vi "set OBW - Sweep Time.vi"(8 "error in (no error)":errorcluster, 9 "Auto?":bool, 10 "Sweep Time (s)":dbl format="%#_6p", 11 "Keysight 9020A in":refnum<class "Keysight 9020A.lvclass">) -> (0 "error out":errorcluster, 3 "Keysight 9020A out":refnum<class "Keysight 9020A.lvclass">)   [LabVIEW 2023, in "Spectrum Analyzer.lvlib" / "Keysight 9020A.lvclass"]
uses:
  Keysight 9020A.lvclass
  Keysight 9020A.lvclass/Keysight 9020A.ctl
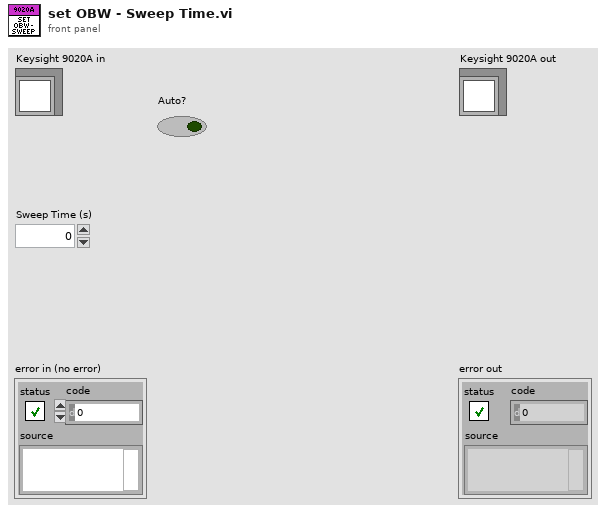
[diagram p1: front panel]
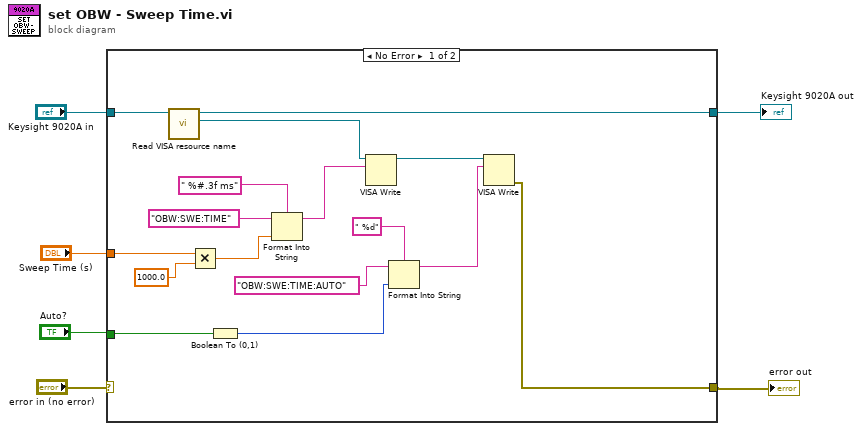
[diagram p0: block diagram]
diagram:
  n1 = case shown="No Error" "error in (no error)" {
    selector: "error in (no error)" -> [_ w23]
    tunnel: "Keysight 9020A in" -> [w22 w24]
    tunnel: [w21 w24] -> w5
    tunnel: [w8 w23] -> w3
    tunnel: "Sweep Time (s)" -> [w18 _]
    tunnel: "Auto?" -> [w10 _]
    frame No Error {
      n2 = call "Read VISA resource name.vi"("Keysight 9020A in"=w22) -> ("VISA resource name"=w7:refnum<visa-resource-name>, "Keysight 9020A out"=w21:refnum<class "Keysight 9020A.lvclass">)  [unwired: 8 in, 1 out]
      n3 = Multiply(x=w18, y=1000.0) -> (x*y=w16:dbl)
      n4 = Boolean To (0,1)(Boolean=w10) -> (0, 1=w9:i16)
      n5 = Format Into String(format string=" %#.3f ms", initial string="OBW:SWE:TIME", w16) -> (resulting string=w19:string)  [unwired: 1 in, 1 out]
      n6 = VISA Write(VISA resource name=w7, write buffer=w19) -> (VISA resource name out=w14:refnum<visa-resource-name>)  [unwired: 1 in, 2 out]
      n7 = Format Into String(format string=" %d", initial string="OBW:SWE:TIME:AUTO", w9) -> (resulting string=w11:string)  [unwired: 1 in, 1 out]
      n8 = VISA Write(VISA resource name=w14, write buffer=w11) -> (error out=w8:errorcluster)  [unwired: 1 in, 2 out]
    }
    frame Error {
    }
  }
  "error out" <- w3
  "Keysight 9020A out" <- w5
